vi "Create User.vi"(5 "Save File":bool=TRUE, 6 "error in (no error)":errorcluster, 7 "Password":string, 8 "LoginName":string, 9 "EasyUserManager in":refnum<class "EasyUserManager.lvclass">) -> (0 "error out":errorcluster, 3 "EasyUserManager out":refnum<class "EasyUserManager.lvclass">)   [LabVIEW 2024, in "EasyUserManager.lvclass"]
doc: "Create a new Teststand User with the provided <B>LoginName</B> and <B>Password</B>. \n\nThe boolean input <B>Save File</B> controls whether changes are immediately saved to the users file (Default: True)."
uses:
  EasyUserManager.lvclass
  EasyUserManager.lvclass/EasyUserManager.ctl
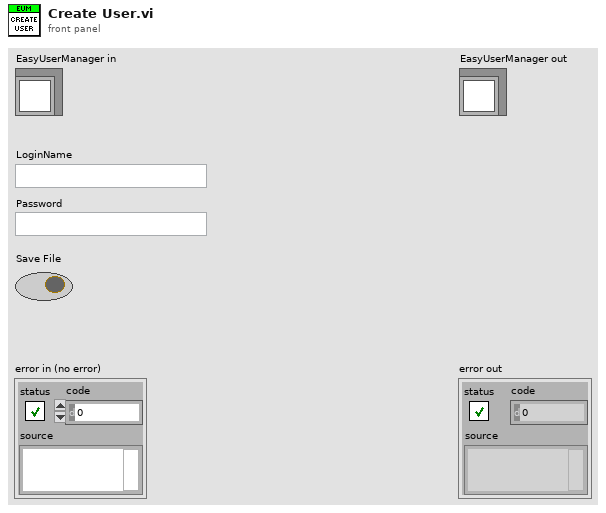
[diagram p1: front panel]
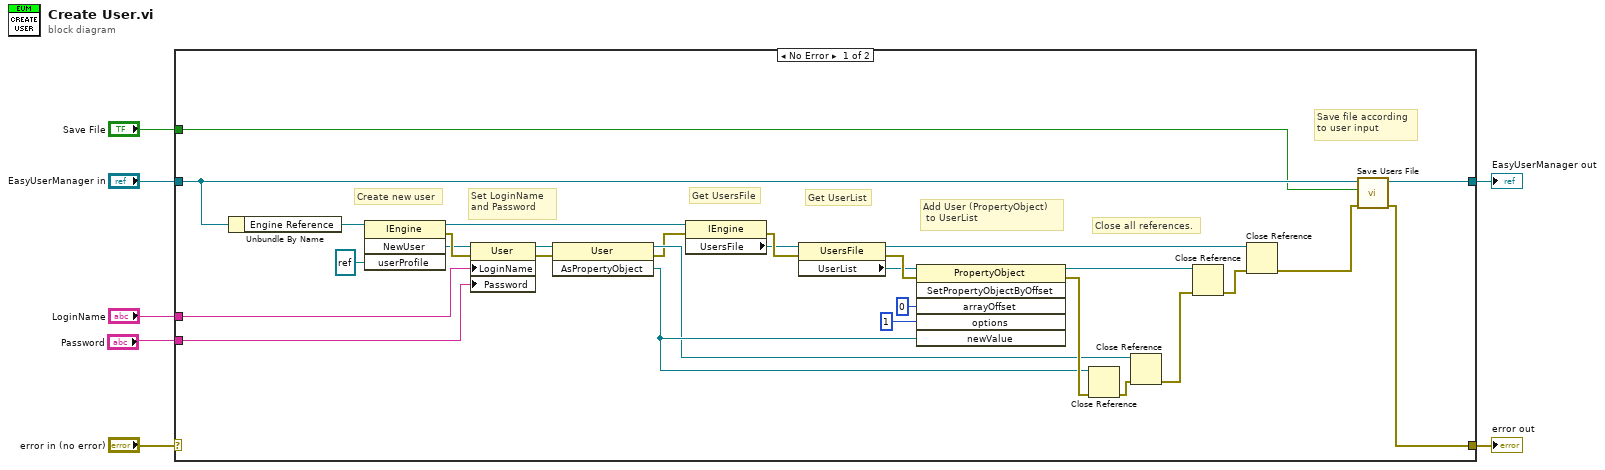
[diagram p0: block diagram]
diagram:
  n1 = case shown="No Error" "error in (no error)" {
    selector: "error in (no error)" -> [_ w38]
    tunnel: [w11 w38] -> w6
    tunnel: [w14 w37] -> w4
    tunnel: "EasyUserManager in" -> [w13 w37]
    tunnel: "Password" -> [w10 _]
    tunnel: "LoginName" -> [w9 _]
    tunnel: "Save File" -> [w8 _]
    frame No Error {
      # "Close all references."
      # "Add User (PropertyObject)\n to UserList"
      # "Get UserList"
      # "Get UsersFile"
      # "Set LoginName \nand Password"
      # "Create new user"
      # "Save file according\nto user input"
      n2 = Unbundle By Name(w13) -> ("Engine Reference"=w15:refnum<k7>)
      n3 = invoke on="Invoke Node" class="IEngine" method="NewUser"(reference=w15, "userProfile"=refnum<k7> refnum) -> (reference out=w21:refnum<k7>, error out=w20:errorcluster, "NewUser"=w19:refnum<k7>)  [unwired: 2 in, 1 out]
      n4 = property on="Property Node" class="User"(reference=w19, error in=w20, "LoginName"=w9, "Password"=w10) -> (reference out=w24:refnum<k7>, error out=w25:errorcluster)
      n5 = invoke on="Invoke Node" class="User" method="AsPropertyObject"(reference=w24, error in=w25) -> (reference out=w29:refnum<k7>, error out=w26:errorcluster, "AsPropertyObject"=w30:refnum<k7>)  [unwired: 1 in]
      n6 = property on="Property Node" class="IEngine"(reference=w21, error in=w26) -> (error out=w27:errorcluster, "UsersFile"=w22:refnum<k7>)  [unwired: 1 out]
      n7 = property on="Property Node" class="UsersFile"(reference=w22, error in=w27) -> (reference out=w36:refnum<k7>, error out=w28:errorcluster, "UserList"=w23:refnum<k7>)
      n8 = invoke on="Invoke Node" class="PropertyObject" method="SetPropertyObjectByOffset"(reference=w23, error in=w28, "arrayOffset"=0, "options"=1, "newValue"=w30) -> (reference out=w34:refnum<k7>, error out=w31:errorcluster)  [unwired: 1 in, 4 out]
      n9 = Close Reference(reference=w30, error in (no error)=w31) -> (error out=w32:errorcluster)
      n10 = Close Reference(reference=w29, error in (no error)=w32) -> (error out=w33:errorcluster)
      n11 = Close Reference(reference=w34, error in (no error)=w33) -> (error out=w35:errorcluster)
      n12 = Close Reference(reference=w36, error in (no error)=w35) -> (error out=w12:errorcluster)
      n13 = call "Save Users File.vi"("error in (no error)"=w12, "Save"=w8, "EasyUserManager in"=w13) -> ("error out"=w11:errorcluster, "EasyUserManager out"=w14:refnum<class "EasyUserManager.lvclass">)  [unwired: 3 in]
    }
    frame Error {
      # "Pass error and do nothing."
    }
  }
  "error out" <- w6
  "EasyUserManager out" <- w4
